vi "Read U64 Direct.vi"(8 "error in (no error)":errorcluster, 11 "CIFTag in":refnum<class "CIF_Iceoryx_Chn_U64.lvclass">) -> (0 "error out":errorcluster, 2 "Data":u64, 3 "CIFTag out":refnum<class "CIF_Iceoryx_Chn_U64.lvclass">)   [LabVIEW 2021, in "CIF_Iceoryx_Chn_U64.lvclass"]
uses:
  CIF_Iceoryx_Chn_U64.lvclass
  CIFChannels/CIFChannels.lvclass/CIFChannels.ctl
  ChannelCommon/typedef/Channel State.ctl
  ChannelCommon/typedef/Direction.ctl
  CIF_Iceoryx_Chn_U64.lvclass/CIF_Iceoryx_Chn_U64.ctl
  CIF_Iceoryx_BB/CIF_Iceoryx_BB.lvclass/CIF_Iceoryx_BB.ctl
  959f43c0-2965-45e0-a797-017a19813e3c.vi
  CIFChannels/Accessors/Read Channel State.vi
  CIFChannels/Accessors/Read Direction.vi
  CIFChannels/Accessors/Read Tag Forced.vi
  <vilib>/CIF Foundation/CIF Iceoryx/SubVIs/Get Path.vi
  <vilib>/CIF Foundation/CIF Iceoryx/SubVIs/Convert Error.vi
  <vilib>/CIF Foundation/CIF Iceoryx/Refnum/BB Reader from Refnum.vi
  <vilib>/CIF Foundation/CIF Iceoryx/SubVIs/Convert Error Core.vi
  ChannelCommon/ChannelCommon.lvlib
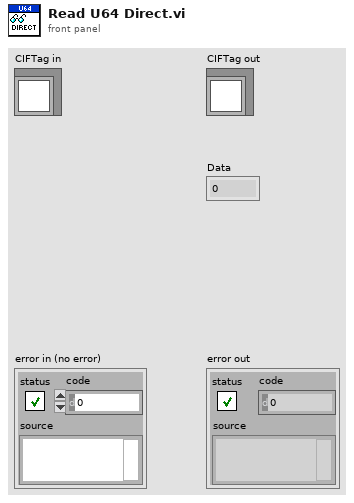
[diagram p1: front panel]
types:
  T1 = typedef "ChannelCommon.lvlib/Channel State.ctl" = enum8{"Creating", "Disconnected", "Connecting", "Connected", "Destroyed"}
  T2 = typedef "ChannelCommon.lvlib/Direction.ctl" = enum8{"Publisher", "Subscriber"}
  T3 = typedef "Iceoryx.lvlib/BB Reader Refnum.ctl" = cluster{"refnum":u64, "BB Reader":enum8{"bb_reader"}}
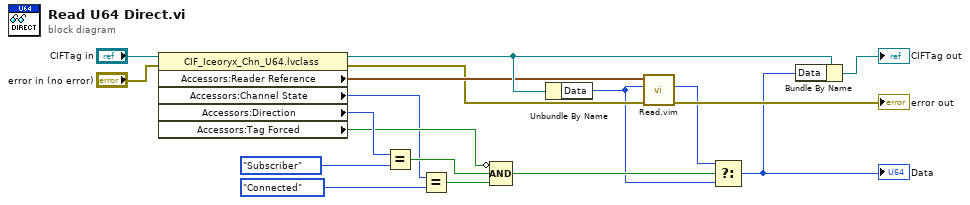
[diagram p0: block diagram]
diagram:
  n1 = property class="CIF_Iceoryx_Chn_U64.lvclass"(reference="CIFTag in", error in="error in (no error)") -> (reference out=w7:refnum<class "CIF_Iceoryx_Chn_U64.lvclass">, error out=w5:errorcluster, "Accessors:Reader Reference"=w6:T3, "Accessors:Channel State"=w8:T1, "Accessors:Direction"=w14:T2, "Accessors:Tag Forced"=w9:bool)
  n2 = Equal?(x=w14, y=Direction."Subscriber") -> (x = y?=w10:bool)
  n3 = Equal?(x=w8, y=Channel_State."Connected") -> (x = y?=w11:bool)
  n4 = Compound Arithmetic op=AND(invert w9, w10, w11) -> (w4:bool)
  n5 = Unbundle By Name(w7) -> ("Data"=w2:u64)
  n6 = call "Read.vim"("error in (no error)"=w5, "Data In"=w2, "Reader Reference"=w6) -> ("error out"=→"error out":errorcluster, "Data Out"=w3:u64)  [unwired: 6 in, 1 out]
  n7 = Select(t=w3, s=w4, f=w2) -> (s? t:f=w1:u64)
  "Data" <- w1
  n8 = Bundle By Name(cluster=w7, "Data"=w1) -> (→"CIFTag out":refnum<class "CIF_Iceoryx_Chn_U64.lvclass">)
